vi "test28-MappingRelationshipByExternalRegistration_API_State.vi"(8 "error in (no error)":errorcluster, 11 "TestCase in":refnum<class "testcase-CSMBroadcast.lvclass">) -> (0 "error out":errorcluster, 3 "TestCase out":refnum<class "testcase-CSMBroadcast.lvclass">)   [LabVIEW 2017, in "testcase-CSMBroadcast.lvclass"]
uses:
  testcase-CSMBroadcast.lvclass
  src/user.lib/_NEVSTOP/Communicable State Machine(CSM)/Communicable State Machine.lvlib
  <vilib>/addons/_JKI Toolkits/VI Tester/TestCase.llb/TestCase.lvclass
  C:/Program Files (x86)/National Instruments/LabVIEW 2017/vi.lib/addons/_JKI Toolkits/VI Tester/TestCase.llb/TestCase.lvclass
panel:
  out "Loop Count":i32
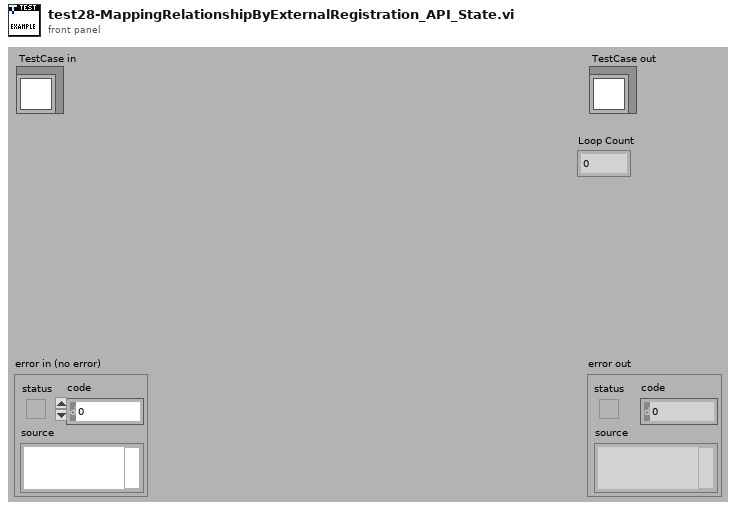
[diagram p1: front panel]
types:
  T1 = cluster{"Status":string, "Source CSM":string, "Target CSM":string, "Target API":string}[]
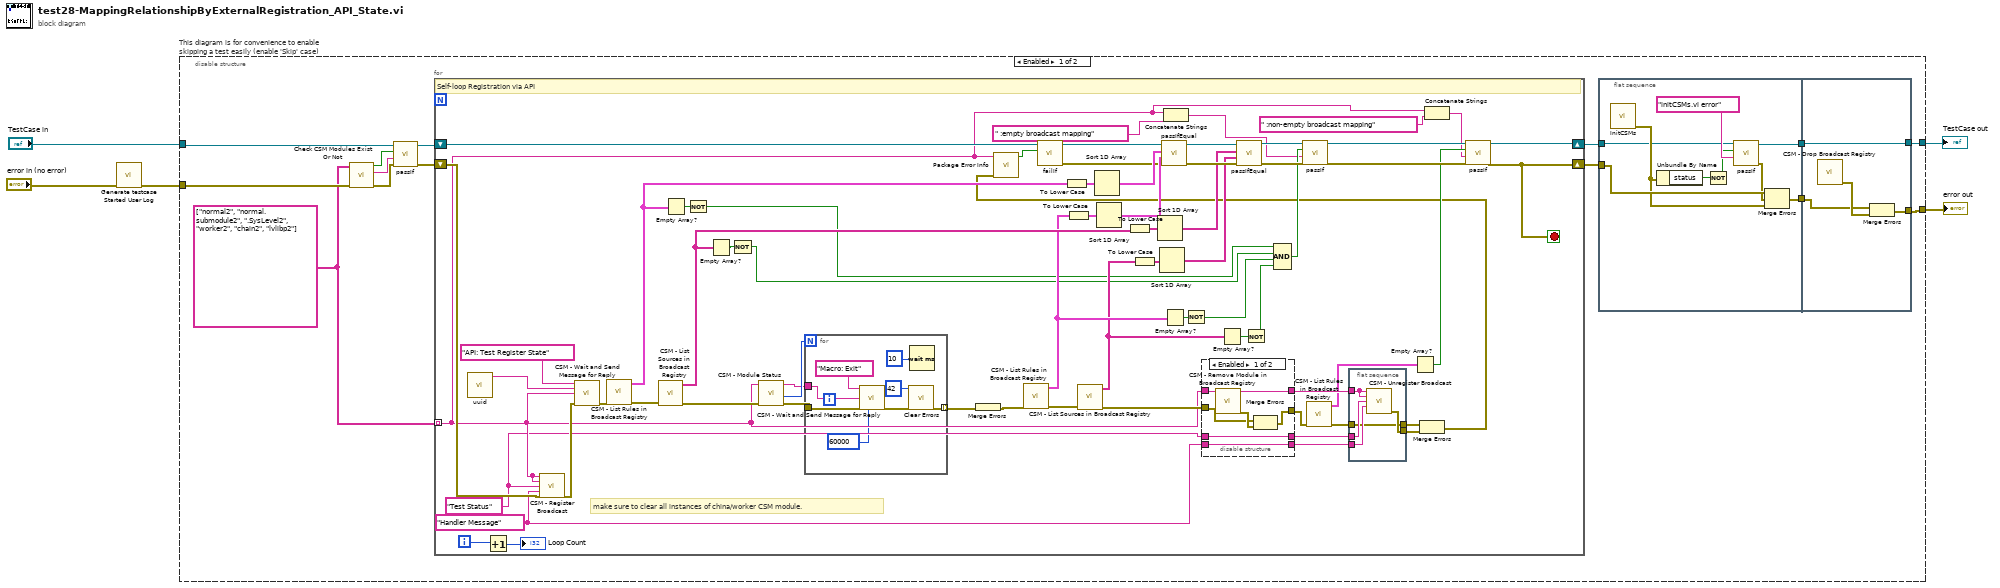
[diagram p0: block diagram]
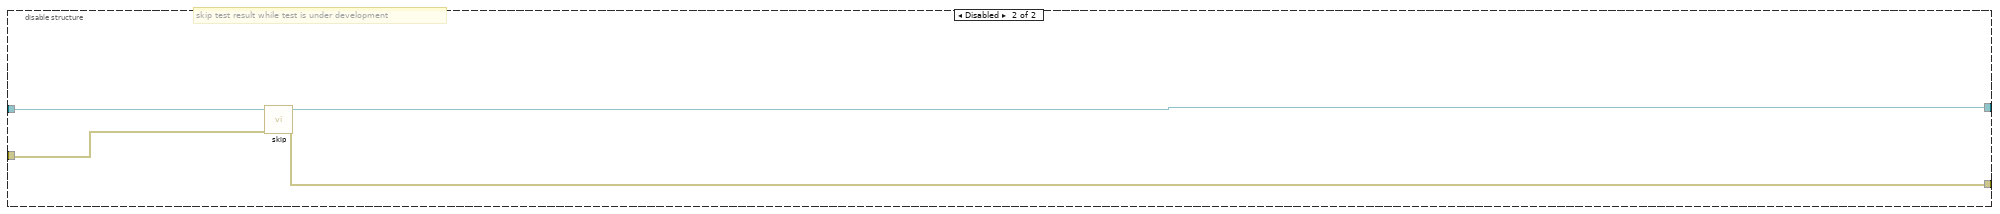
[diagram p3: hidden frame]
diagram:
  n1 = call "Generate testcase Started User Log.vi"("Error In"="error in (no error)") -> ("error out"=w1:errorcluster)  [unwired: 10 in]
  n2 = disable-structure "This diagram is for convenience to enable skipping a test easily (enable 'Skip' case)" shown="Enabled" {
    disable-tunnel: "TestCase in" -> [w16 w126]
    disable-tunnel: [w7 w124] -> w2
    disable-tunnel: [w6 w125] -> w4
    disable-tunnel: w1 -> [w13 w123]
    frame Enabled {
      w12 = string[] ["normal2", "normal.submodule2", ".SysLevel2", "worker2", "chain2", "lvlibp2"]
      n3 = call "Check CSM Modules Exist Or Not.vi"("error in"=w13, "CSM names in"=w12) -> ("error out"=w17:errorcluster, "Debug string"=w18:string, "All Modules Exist?"=w19:bool)  [unwired: 7 in]
      n4 = call-dynamic "passIf.vi"("error in (no error)"=w17, "message (\"\")"=w18, "pass"=w19, "TestCase in"=w16) -> ("error out"=w14:errorcluster, "TestCase out"=w15:refnum<class "testcase-CSMBroadcast.lvclass">)  [unwired: 6 in]
      n5 = for {
        tunnel: w12 -> [w35] mode=indexing
        shift-right: [w62] -> w9
        shift-left: w15 -> [w52]
        shift-right: [w58] -> w8
        shift-left: w14 -> [w59]
        i -> [w81]
        stop <- w58 stop-if-true
        w33 = "Handler Message" ("Response Message (If \"\", Same as Source Message)")
        w34 = "Test Status" ("Status")
        # "make sure to clear all instances of china/worker CSM module."
        # "Self-loop Registration via API"
        n6 = call "uuid.vi"() -> ("UUID"=w97:string)  [unwired: 11 in]
        n7 = Increment(x=w81) -> (x+1=→"Loop Count":i32)
        n8 = call "CSM - Register Broadcast.vi"("CSM Name(Empty for Broadcast Event)"=w35, "Source CSM Name (* as Default)"=w35, "Trigger"=w34, "API (If \"\", Same as Trigger)"=w33, "Error In"=w59) -> ("error out"=w64:errorcluster)  [unwired: 9 in, 1 out]
        n9 = call "CSM - Wait and Send Message for Reply.vi"("State"="API: Test Register State", "Arguments (\"\")"=w97, "Target Module"=w35, "Error In (No Error)"=w64) -> ("error out"=w96:errorcluster)  [unwired: 8 in, 3 out]
        n10 = call "CSM - List Rules in Broadcast Registry.vi"("error in (no error)"=w96) -> ("error out"=w93:errorcluster, "Rule Entries"=w79:T1)  [unwired: 8 in, 1 out]
        n11 = call "CSM - List Sources in Broadcast Registry.vi"("error in (no error)"=w93) -> ("error out"=w54:errorcluster, "Broadcast Names"=w76:string[])  [unwired: 9 in]
        n12 = Empty Array?(array=w79) -> (empty?=w78:bool)
        n13 = Not(x=w78) -> (.not. x?=w71:bool)
        n14 = Empty Array?(array=w76) -> (empty?=w77:bool)
        n15 = Not(x=w77) -> (.not. x?=w70:bool)
        n16 = call "CSM - Module Status.vi"("Error In"=w54, "CSM Name"=w35) -> ("error out"=w55:errorcluster, "#Nodes"=w57:i32, "CSM Name (Dup)"=w56:string)  [unwired: 5 in, 2 out]
        n17 = for {
          N: w57 -> [_]
          tunnel: w56 -> [w120]
          tunnel: w55 -> [w119]
          tunnel: [w118] -> w95 mode=indexing
          n18 = call "CSM - Wait and Send Message for Reply.vi"("State"="Macro: Exit", "Target Module"=w120, "Error In (No Error)"=w119, "Response Timeout (-2 Using Global Settings)"=60000) -> ("error out"=w121:errorcluster)  [unwired: 8 in, 3 out]
          n19 = call <vilib>:"Clear Errors.vi"("error in (no error)"=w121, "specific error code to clear (0: all)"=42) -> ("error out"=w118:errorcluster)  [unwired: 4 in, 1 out]
          n20 = Wait (ms)(milliseconds to wait=u32 10) -> ()  [unwired: 1 out]
        }
        n21 = Merge Errors(w95) -> (w94:errorcluster)
        n22 = call "CSM - List Rules in Broadcast Registry.vi"("error in (no error)"=w94) -> ("error out"=w92:errorcluster, "Rule Entries"=w74:T1)  [unwired: 8 in, 1 out]
        n23 = To Lower Case(string=w79) -> (all lower case string=w91:T1)
        n24 = To Lower Case(string=w74) -> (all lower case string=w90:T1)
        n25 = call "CSM - List Sources in Broadcast Registry.vi"("error in (no error)"=w92) -> ("error out"=w38:errorcluster, "Broadcast Names"=w72:string[])  [unwired: 9 in]
        n26 = Sort 1D Array(array=w91) -> (sorted array=w89:T1)
        n27 = Sort 1D Array(array=w90) -> (sorted array=w88:T1)
        n28 = To Lower Case(string=w76) -> (all lower case string=w85:string[])
        n29 = To Lower Case(string=w72) -> (all lower case string=w84:string[])
        n30 = Sort 1D Array(array=w85) -> (sorted array=w83:string[])
        n31 = Sort 1D Array(array=w84) -> (sorted array=w82:string[])
        n32 = Empty Array?(array=w74) -> (empty?=w75:bool)
        n33 = Concatenate Strings(w35, " :empty broadcast mapping" ("string")) -> (w47:string)
        n34 = Not(x=w75) -> (.not. x?=w69:bool)
        n35 = disable-structure shown="Enabled" {
          disable-tunnel: w38 -> [w104 w113]
          disable-tunnel: [w108 w113] -> w44
          disable-tunnel: w35 -> [w109 w114]
          disable-tunnel: w34 -> [w106 w112]
          disable-tunnel: w33 -> [w105 w111]
          disable-tunnel: [w107 w114] -> w45
          disable-tunnel: [w106 w112] -> w43
          disable-tunnel: [w105 w111] -> w42
          frame Enabled {
            n36 = call "CSM - Remove Module in Broadcast Registry.vi"("CSM Name"=w109) -> ("CSM Name (Dup)"=w107:string, "error out"=w110:errorcluster)  [unwired: 13 in]
            n37 = Merge Errors(w104, w110) -> (w108:errorcluster)
          }
          frame Disabled {
          }
        }
        n38 = Empty Array?(array=w72) -> (empty?=w73:bool)
        n39 = Not(x=w73) -> (.not. x?=w68:bool)
        n40 = Compound Arithmetic op=AND(w71, w70, w69, w68) -> (w65:bool)
        n41 = call "CSM - List Rules in Broadcast Registry.vi"("error in (no error)"=w44) -> ("error out"=w40:errorcluster, "Rule Entries"=w36:T1)  [unwired: 8 in, 1 out]
        n42 = flat-sequence {
          tunnel: w45 -> [w103]
          tunnel: w43 -> [w102]
          tunnel: w42 -> [w101]
          tunnel: [w100] -> w41
          tunnel: w40 -> [w99]
          tunnel: [w99] -> w39
          frame #0 {
            n43 = call "CSM - Unregister Broadcast.vi"("CSM Name(Empty for Broadcast Event)"=w103, "Source CSM Name (* as Default)"=w103, "Trigger"=w102, "API (\"*\" as Default)"=w101) -> ("error out"=w100:errorcluster)  [unwired: 10 in, 1 out]
          }
        }
        n44 = Empty Array?(array=w36) -> (empty?=w60:bool)
        n45 = Merge Errors(w39, w41) -> (w37:errorcluster)
        n46 = call "Package Error Info.vi"("error in"=w37, "String in"=w35) -> ("error status"=w53:bool)  [unwired: 8 in, 1 out]
        n47 = call-dynamic "failIf.vi"("fail"=w53, "TestCase in"=w52) -> ("error out"=w50:errorcluster, "TestCase out"=w51:refnum<class "testcase-CSMBroadcast.lvclass">)  [unwired: 8 in]
        n48 = call-dynamic "passIfEqual.vi"("error in (no error)"=w50, "y"=w88, "x"=w89, "TestCase in"=w51) -> ("error out"=w86:errorcluster, "TestCase out"=w87:refnum<class "testcase-CSMBroadcast.lvclass">)  [unwired: 6 in]
        n49 = call-dynamic "passIfEqual.vi"("error in (no error)"=w86, "y"=w82, "x"=w83, "TestCase in"=w87) -> ("error out"=w66:errorcluster, "TestCase out"=w67:refnum<class "testcase-CSMBroadcast.lvclass">)  [unwired: 6 in]
        n50 = call-dynamic "passIf.vi"("error in (no error)"=w66, "message (\"\")"=w47, "pass"=w65, "TestCase in"=w67) -> ("error out"=w61:errorcluster, "TestCase out"=w63:refnum<class "testcase-CSMBroadcast.lvclass">)  [unwired: 6 in]
        n51 = Concatenate Strings(w35, " :non-empty broadcast mapping" ("string")) -> (w46:string)
        n52 = call-dynamic "passIf.vi"("error in (no error)"=w61, "message (\"\")"=w46, "pass"=w60, "TestCase in"=w63) -> ("error out"=w58:errorcluster, "TestCase out"=w62:refnum<class "testcase-CSMBroadcast.lvclass">)  [unwired: 6 in]
      }
      n53 = flat-sequence {
        tunnel: w9 -> [w20]
        tunnel: [w28] -> w11
        tunnel: w8 -> [w25]
        tunnel: [w22] -> w10
        tunnel: w11 -> [w31]
        tunnel: [w31] -> w7
        tunnel: [w30] -> w6
        tunnel: w10 -> [w29]
        frame #0 {
          n54 = call "InitCSMs.vi"() -> ("error out"=w23:errorcluster)  [unwired: 10 in, 1 out]
          n55 = Unbundle By Name(w23) -> ("status"=w27:bool)
          n56 = Not(x=w27) -> (.not. x?=w21:bool)
          n57 = call-dynamic "passIf.vi"("message (\"\")"="initCSMs.vi error" ("message (\"\")"), "pass"=w21, "TestCase in"=w20) -> ("error out"=w24:errorcluster, "TestCase out"=w28:refnum<class "testcase-CSMBroadcast.lvclass">)  [unwired: 7 in]
          n58 = Merge Errors(w25, w24, w23) -> (w22:errorcluster)
        }
        frame #1 {
          n59 = call "CSM - Drop Broadcast Registry.vi"() -> ("error out"=w32:errorcluster)  [unwired: 15 in]
          n60 = Merge Errors(w29, w32) -> (w30:errorcluster)
        }
      }
    }
    frame Disabled {
      # "skip test result while test is under development"
      n61 = call <vilib>:"skip.vi"("error in (no error)"=w123, "TestCase in"=w126) -> ("error out"=w125:errorcluster, "TestCase out"=w124:refnum<class "testcase-CSMBroadcast.lvclass">)  [unwired: 8 in]
    }
  }
  "error out" <- w4
  "TestCase out" <- w2
